vi "VIH ProjFile - Load.vi"(8 "error in":errorcluster, 11 "Project File Path":path) -> (0 "error out":errorcluster, 3 "Project":T1)   [LabVIEW 2014]
doc: "::: VI Helpeks :::\nCopyright (c) 2000-2026 Konstantin Shifershteyn. All rights reserved."
uses:
  <vilib>/xml/Close Reference(Node).vi
  <vilib>/xml/NI_XML.lvlib
  <resource>/objmgr/DOMUserDefRef.rc
panel:
  # "VI Helpeks\nCopyright (c) 2012-2026 Konstantin Shifershteyn"
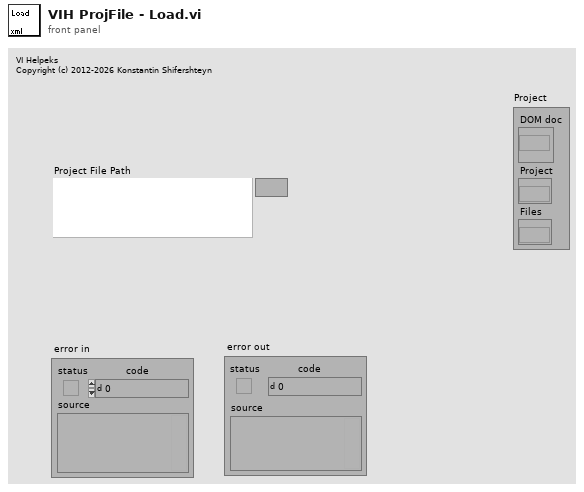
[diagram p1: front panel]
types:
  T1 = cluster{"DOM doc":refnum<k20>, "Project":refnum<k20>, "Files":refnum<k20>}
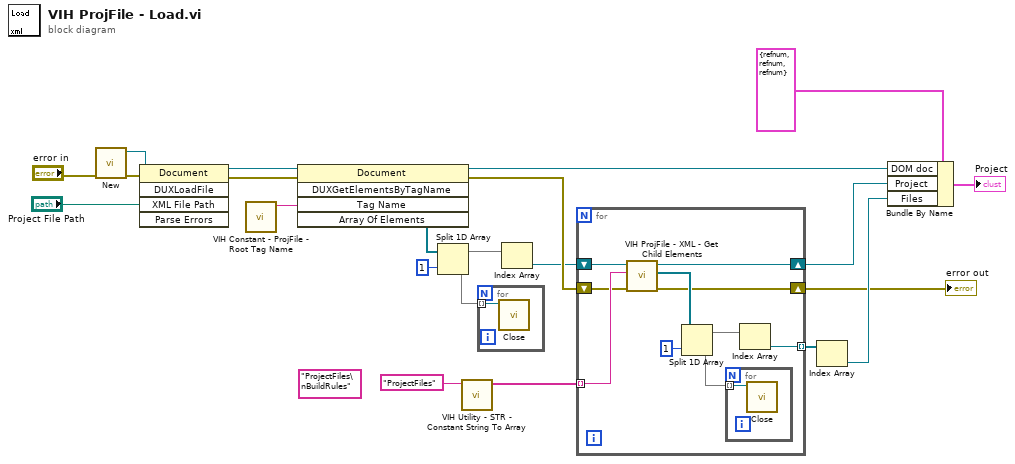
[diagram p0: block diagram]
diagram:
  (unwired) "ProjectFiles\nBuildRules" ("Tag Name")
  n1 = call <vilib>:"New.vi"("error in (no error)"="error in") -> ("error out"=w21:errorcluster, "DOM document out"=w22:refnum<k20>)  [unwired: 7 in]
  n2 = invoke class="Document" method="DUXLoadFile"(reference=w22, error in=w21, "XML File Path"="Project File Path") -> (reference out=w3:refnum<k20>, error out=w20:errorcluster)  [unwired: 2 in, 3 out]
  n3 = call "VIH Constant - ProjFile - Root Tag Name.vi"() -> ("Tag Name"=w1:string)  [unwired: 11 in]
  n4 = invoke class="Document" method="DUXGetElementsByTagName"(reference=w3, error in=w20, "Tag Name"=w1) -> (reference out=w18:refnum<k20>, error out=w14:errorcluster, "Array Of Elements"=w11:refnum<k20>[])  [unwired: 2 in, 2 out]
  n5 = Split 1D Array(array=w11, index=1) -> (first subarray=w9:refnum<k20>[], second subarray=w7:refnum<k20>[])
  n6 = call "VIH Utility - STR - Constant String To Array.vi"("String in"="ProjectFiles" ("Tag Name")) -> ("Array out"=w4:string[])  [unwired: 10 in]
  n7 = for {
    tunnel: w7 -> [w23] mode=indexing
    n8 = call-poly <vilib>:"Close.vi"("node"=w23) -> ()  [unwired: 8 in, 1 out]
  }
  n9 = Index Array(array=w9) -> (element=w8:refnum<k20>)  [unwired: 1 in]
  n10 = for {
    tunnel: w4 -> [w28] mode=indexing
    tunnel: [w31] -> w16 mode=indexing
    shift-right: [w25] -> w12
    shift-left: w14 -> [w26]
    shift-right: [w24] -> w2
    shift-left: w8 -> [w29]
    n11 = call "VIH ProjFile - XML - Get Child Elements.vi"("error in"=w26, "Tag Name"=w28, "XML Parent Item"=w29) -> ("error out"=w25:errorcluster, "Array of Elements"=w27:refnum<k20>[], "dup XML Parent Item"=w24:refnum<k20>)  [unwired: 6 in]
    n12 = Split 1D Array(array=w27, index=1) -> (first subarray=w30:refnum<k20>[], second subarray=w32:refnum<k20>[])
    n13 = for {
      tunnel: w32 -> [w34] mode=indexing
      n14 = call-poly <vilib>:"Close.vi"("node"=w34) -> ()  [unwired: 8 in, 1 out]
    }
    n15 = Index Array(array=w30) -> (element=w31:refnum<k20>)  [unwired: 1 in]
  }
  "error out" <- w12
  n16 = Index Array(array=w16) -> (element=w15:refnum<k20>)  [unwired: 1 in]
  n17 = Bundle By Name(cluster=T1 {"DOM doc"=refnum, "Project"=refnum, "Files"=refnum} ("Project"), "DOM doc"=w18, "Project"=w2, "Files"=w15) -> (→"Project":T1)
